vi "Save to File.vi"(8 "error in":errorcluster, 10 "Folder":path, 11 "ILabVIEWFile in":refnum<class "LabVIEW File.lvclass">) -> (0 "error out":errorcluster, 2 "File Path":path, 3 "ILabVIEWFile out":refnum<class "LabVIEW File.lvclass">)   [LabVIEW 2026, in "LabVIEW File.lvclass"]
doc: "Save object to file at the provided path."
uses:
  LabVIEW File.lvclass
  LabVIEW File.lvclass/LabVIEW File.ctl
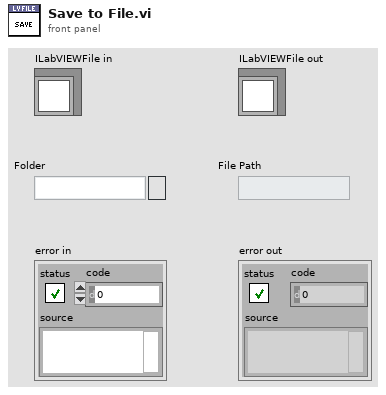
[diagram p1: front panel]
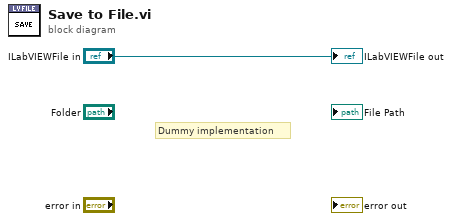
[diagram p0: block diagram]
diagram:
  # "Dummy implementation"
  "ILabVIEWFile out" <- "ILabVIEWFile in"
